vi "Initialize RxTx.vi"(8 "error in (no error)":errorcluster, 10 "Remote IP":string="200.131.64.49", 11 "Filter_Wheel in":refnum<class "Filter_Wheel.lvclass">) -> (0 "error out":errorcluster, 3 "Filter_Wheel out":refnum<class "Filter_Wheel.lvclass">)   [LabVIEW 2018, in "Filter_Wheel.lvclass"]
uses:
  Filter_Wheel.lvclass
  Filter_Wheel.lvclass/Filter_Wheel.ctl
  RxTx/RxTx.lvclass
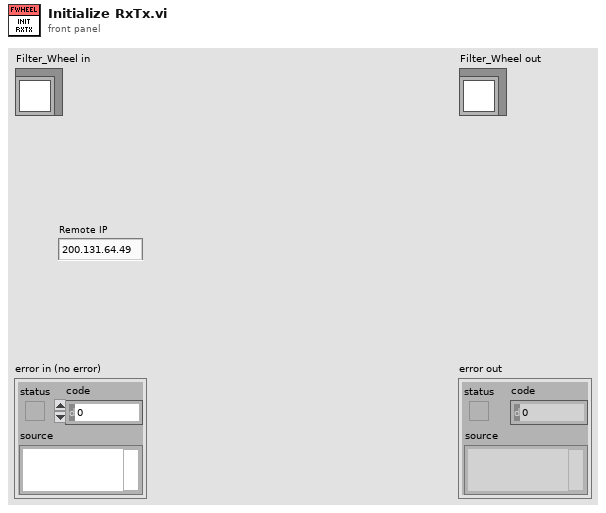
[diagram p1: front panel]
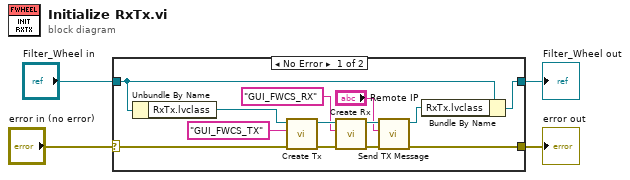
[diagram p0: block diagram]
diagram:
  n1 = case shown="No Error" "error in (no error)" {
    selector: "error in (no error)" -> [w15 w19]
    tunnel: [w7 w19] -> w3
    tunnel: [w16 w18] -> w1
    tunnel: "Filter_Wheel in" -> [w17 w18]
    frame No Error {
      n2 = Unbundle By Name(w17) -> ("RxTx.lvclass"=w12:refnum<class "RxTx.lvclass">)
      n3 = call "Create Tx.vi"("error in (no error)"=w15, "Writer Name"="GUI_FWCS_TX", "RxTx in"=w12) -> ("error out"=w14:errorcluster, "RxTx out"=w13:refnum<class "RxTx.lvclass">)  [unwired: 7 in]
      n4 = call "Create Rx.vi"("error in (no error)"=w14, "Reader Name"="GUI_FWCS_RX" ("Writer Name"), "RxTx in"=w13) -> ("error out"=w6:errorcluster, "RxTx out"=w9:refnum<class "RxTx.lvclass">)  [unwired: 7 in]
      n5 = call "Send TX Message.vi"("error in (no error)"=w6, "element"="Remote IP", "RxTx in"=w9) -> ("error out"=w7:errorcluster, "RxTx out"=w8:refnum<class "RxTx.lvclass">)  [unwired: 7 in]
      n6 = Bundle By Name(cluster=w17, "RxTx.lvclass"=w8) -> (w16:refnum<class "Filter_Wheel.lvclass">)
    }
    frame Error {
    }
  }
  "error out" <- w3
  "Filter_Wheel out" <- w1
